vi "Common.vi"(9 "Action":T1=enum."TemplatesFolderName") -> (1 "Output":string)   [LabVIEW 2020, in "NIVS_Consolidated_CDW_MetaDataObj.lvclass"]
doc: "Contains all constants, which are not part of specific part of the wizard."
uses:
  NIVS_Consolidated_CDW_MetaDataObj.lvclass
  Common.ctl
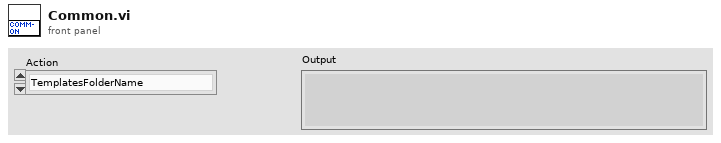
[diagram p1: front panel]
types:
  T1 = typedef "NIVS_Consolidated_CDW_MetaDataObj.lvclass/Common.ctl" = enum16{"ProjectName", "TemplatesFolderName", "PPLTemplatesFolderName", "ProjectTemplatePathAndName", "ProjectPPLTemplatePathAndName", "TimingAndSyncFolderName", "CustomDeviceFolderName", "PathToTemplates", "PathToPPLTemplates", "PathToExplorerPPLTemplates", "PathToEnginePPLTemplates", "PathToConfigurationFile", "ProjectConfigurationName"}
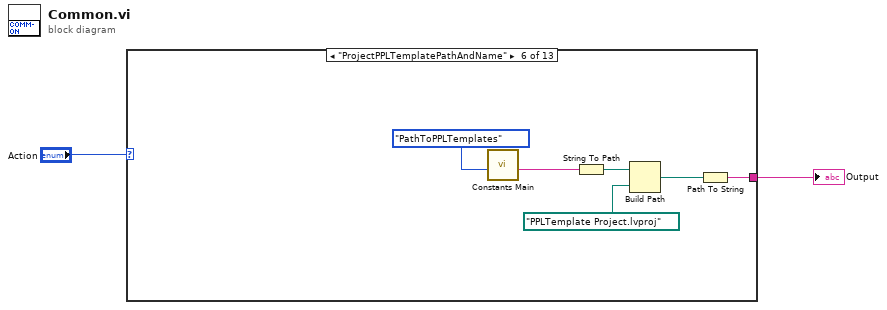
[diagram p0: block diagram]
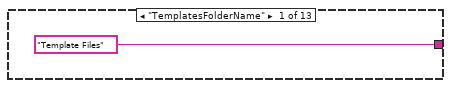
[diagram p2: hidden frame]
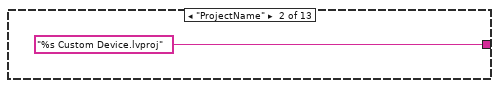
[diagram p3: hidden frame]
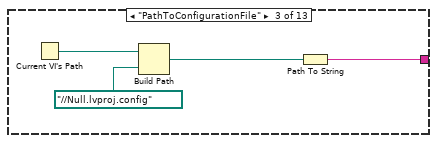
[diagram p4: hidden frame]
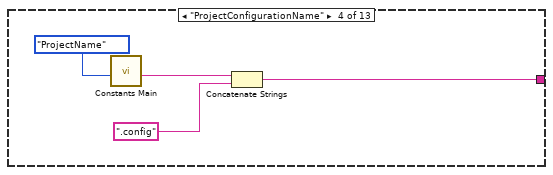
[diagram p5: hidden frame]
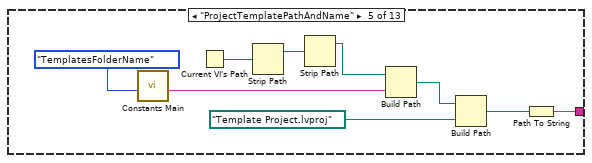
[diagram p6: hidden frame]
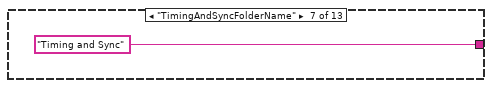
[diagram p7: hidden frame]
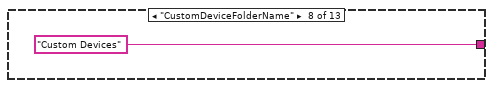
[diagram p8: hidden frame]
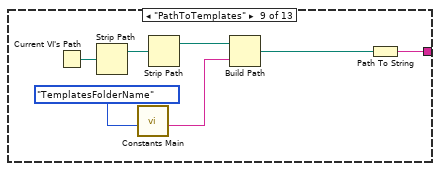
[diagram p9: hidden frame]
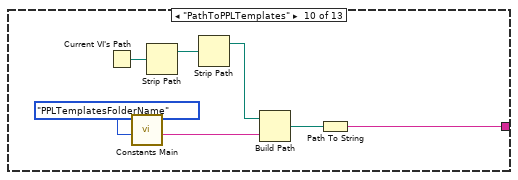
[diagram p10: hidden frame]
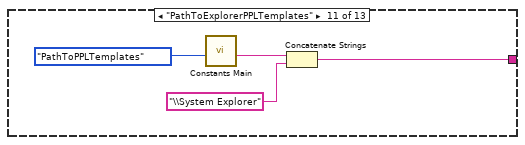
[diagram p11: hidden frame]
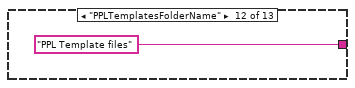
[diagram p12: hidden frame]
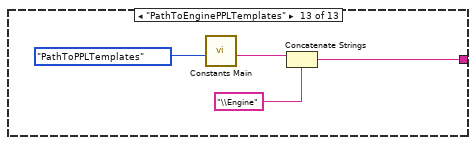
[diagram p13: hidden frame]
diagram:
  n1 = case shown="\"ProjectPPLTemplatePathAndName\"" "Action" {
    tunnel: ["Template Files" "%s Custom Device.lvproj" w8 w9 w16 w24 "Timing and Sync" "Custom Devices" w30 w37 w44 "PPL Template files" w49] -> w2
    frame "TemplatesFolderName" {
    }
    frame "ProjectName" {
    }
    frame "PathToConfigurationFile" {
      n2 = Current VI's Path() -> (path=w6:path)
      n3 = Build Path(base path=w6, name or relative path=path "../../Null.lvproj.config") -> (appended path=w7:path)
      n4 = Path To String(path=w7) -> (string=w8:string)
    }
    frame "ProjectConfigurationName" {
      n5 = call-poly "Constants Main.vi"("Action"=Common."ProjectName") -> ("Output"=w11:string)  [unwired: 10 in]
      n6 = Concatenate Strings(w11, ".config") -> (w9:string)
    }
    frame "ProjectTemplatePathAndName" {
      n7 = call-poly "Constants Main.vi"("Action"=Common."TemplatesFolderName") -> ("Output"=w21:string)  [unwired: 10 in]
      n8 = Current VI's Path() -> (path=w15:path)
      n9 = Strip Path(path=w15) -> (stripped path=w14:path)  [unwired: 1 out]
      n10 = Strip Path(path=w14) -> (stripped path=w13:path)  [unwired: 1 out]
      n11 = Build Path(base path=w13, name or relative path=w21) -> (appended path=w20:path)
      n12 = Build Path(base path=w20, name or relative path=path "Template Project.lvproj") -> (appended path=w18:path)
      n13 = Path To String(path=w18) -> (string=w16:string)
    }
    frame "ProjectPPLTemplatePathAndName" {
      n14 = call-poly "Constants Main.vi"("Action"=Common."PathToPPLTemplates") -> ("Output"=w23:string)  [unwired: 10 in]
      n15 = String To Path(string=w23) -> (path=w22:path)
      n16 = Build Path(base path=w22, name or relative path=path "PPLTemplate Project.lvproj") -> (appended path=w26:path)
      n17 = Path To String(path=w26) -> (string=w24:string)
    }
    frame "TimingAndSyncFolderName" {
    }
    frame "CustomDeviceFolderName" {
    }
    frame "PathToTemplates" {
      n18 = Current VI's Path() -> (path=w33:path)
      n19 = Strip Path(path=w33) -> (stripped path=w32:path)  [unwired: 1 out]
      n20 = call-poly "Constants Main.vi"("Action"=Common."TemplatesFolderName") -> ("Output"=w36:string)  [unwired: 10 in]
      n21 = Strip Path(path=w32) -> (stripped path=w31:path)  [unwired: 1 out]
      n22 = Build Path(base path=w31, name or relative path=w36) -> (appended path=w35:path)
      n23 = Path To String(path=w35) -> (string=w30:string)
    }
    frame "PathToPPLTemplates" {
      n24 = Current VI's Path() -> (path=w40:path)
      n25 = call-poly "Constants Main.vi"("Action"=Common."PPLTemplatesFolderName") -> ("Output"=w43:string)  [unwired: 10 in]
      n26 = Strip Path(path=w40) -> (stripped path=w39:path)  [unwired: 1 out]
      n27 = Strip Path(path=w39) -> (stripped path=w38:path)  [unwired: 1 out]
      n28 = Build Path(base path=w38, name or relative path=w43) -> (appended path=w42:path)
      n29 = Path To String(path=w42) -> (string=w37:string)
    }
    frame "PathToExplorerPPLTemplates" {
      n30 = call-poly "Constants Main.vi"("Action"=Common."PathToPPLTemplates") -> ("Output"=w46:string)  [unwired: 10 in]
      n31 = Concatenate Strings(w46, "\\System Explorer" ("string")) -> (w44:string)
    }
    frame "PPLTemplatesFolderName" {
    }
    frame "PathToEnginePPLTemplates" {
      n32 = call-poly "Constants Main.vi"("Action"=Common."PathToPPLTemplates") -> ("Output"=w51:string)  [unwired: 10 in]
      n33 = Concatenate Strings(w51, "\\Engine" ("string")) -> (w49:string)
    }
  }
  "Output" <- w2
